vi "Keyboard Test.vi"() -> ()   [LabVIEW 2014]
panel:
  in  "stop":bool
  in  "Speed value":dbl=1.0
  out "Control cluster":T1 {"Roll" scale=-1.0..1.0; "Pitch" scale=-1.0..1.0; "Vertical Speed" scale=-1.0..1.0; "Yaw Speed" scale=-1.0..1.0}
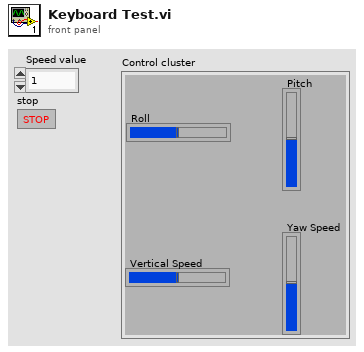
[diagram p1: front panel]
types:
  T1 = cluster{"Roll":dbl, "Pitch":dbl, "Vertical Speed":dbl, "Yaw Speed":dbl}
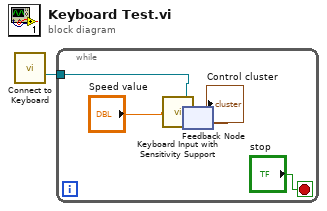
[diagram p0: block diagram]
diagram:
  n1 = call "Connect to Keyboard.vi"() -> ("device ID"=w1:refnum<k1>)  [unwired: 13 in, 2 out]
  n2 = while {
    tunnel: w1 -> [w2]
    stop <- "stop" stop-if-true
    n3 = feedback #1() -> (w4:T1)  [unwired: 1 in]
    "Control cluster" <- w4
    n4 = call "Keyboard Input with Sensitivity Support.vi"("device ID"=w2, "Previous Control Cluster"=w4, "Speed step"="Speed value") -> ("Control Cluster"=w5:T1)  [unwired: 1 in, 1 out]
    n5 = feedback-in #1(w5) -> ()
  }
